vi "Apply Deviation.vi"(8 "error in (no error)":errorcluster, 11 "Tool Path in":refnum<class "Tool Path.lvclass">) -> (0 "error out":errorcluster, 3 "Tool Path out":refnum<class "Tool Path.lvclass">)   [LabVIEW 2019, in "Tool Path.lvclass"]
uses:
  Tool Path.lvclass
  subVIs/typedefs/Schedule Types/Schedule--Formula.ctl
  Settings/Path Settings/Path Settings.lvclass/Path Settings.ctl
  Settings/Path Settings/Path Settings.lvclass
  Settings/ObjectSettings/ObjectSettings.lvclass
  <vilib>/gmath/NI_Gmath.lvlib
  Tool Object/Tool Object.lvclass
panel:
  out "XY Graph":T1(graph)
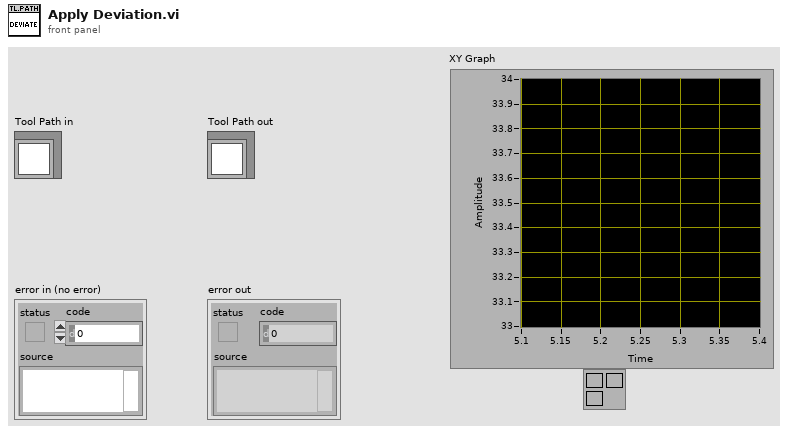
[diagram p1: front panel]
types:
  T1 = cluster{"Resampled X":dbl[], "Resampled Y":dbl[]}[]
  T2 = typedef "Schedule--Formula.ctl" = cluster{"formula":string, "formula length (nm)":dbl, "formula resolution (nm)":dbl}
  T3 = cluster{"Resampled X":dbl[], "Resampled Y":dbl[]}
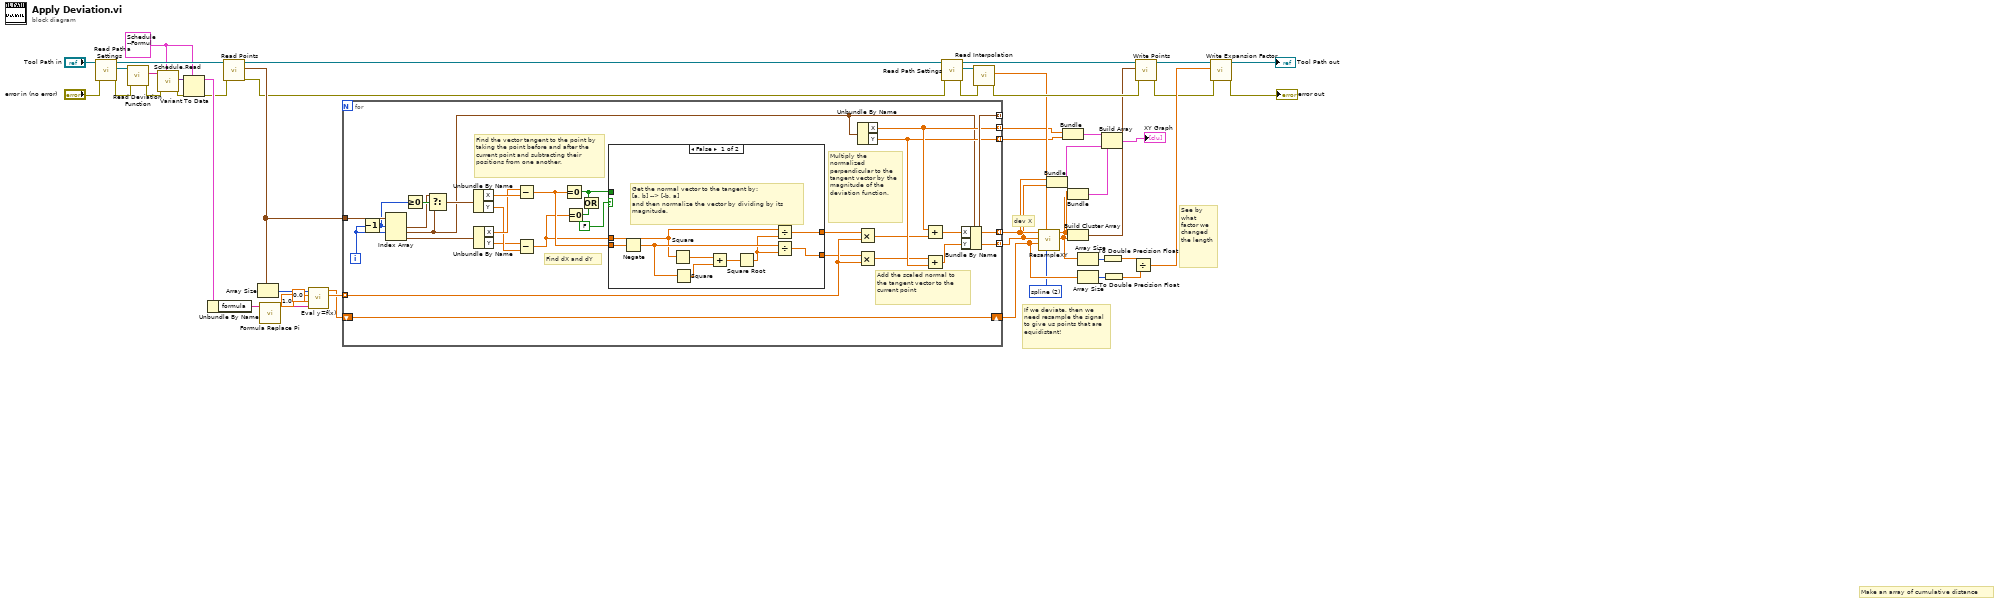
[diagram p0: block diagram]
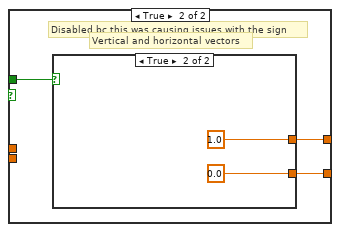
[diagram p2: hidden frame]
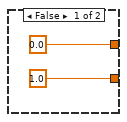
[diagram p3: hidden frame]
diagram:
  w1 = 2 items=["nearest", "linear", "spline", "cubic Hermite", "Lagrange"] ("Interpolation Method")
  w39 = T2 {"formula"="1*(step(170-t)*cos(0.62831853071*t)+step(t-170)*cos(0.62831853071*(t-170))*(-1))", "formula length (nm)"=340.0, "formula resolution (nm)"=0.001} ("Formula")
  # "See by what factor we changed the length"
  # "If we deviate, then we need resample the signal to give us points that are equidistant!"
  # "dev X"
  # "Make an array of cumulative distance"
  n1 = call-dynamic "Read Path Settings.vi"("error in (no error)"="error in (no error)", "Tool Path in"="Tool Path in") -> ("error out"=w38:errorcluster, "Path Settings.lvclass"=w48:refnum<class "Path Settings.lvclass">, "Tool Path out"=w42:refnum<class "Tool Path.lvclass">)  [unwired: 7 in]
  n2 = call-dynamic "Read Deviation Function.vi"("error in (no error)"=w38, "Path Settings in"=w48) -> ("error out"=w28:errorcluster, "Deviation Function"=w45:string)  [unwired: 7 in, 1 out]
  n3 = call "Schedule.Read.vi"("Data to Read"=w39, "error in (no error)"=w28, "Schedule <JSON> In"=w45) -> ("error out"=w44:errorcluster, "Data Out"=w47:variant)  [unwired: 6 in, 1 out]
  n4 = Variant To Data(error in=w44, type=w39, Variant=w47) -> (data=w46:T2, error out=w37:errorcluster)
  n5 = Unbundle By Name(w46) -> ("formula"=w26:string)
  n6 = call-dynamic "Read Points.vi"("error in (no error)"=w37, "Tool Object in"=w42) -> ("error out"=w29:errorcluster, "Points"=w33:cluster{"X":dbl, "Y":dbl}[], "Tool Object out"=w30:refnum<class "Tool Path.lvclass">)  [unwired: 7 in]
  n7 = Array Size(array=w33) -> (size(s)=w34:i32)
  n8 = call "Formula Replace Pi.vi"("Formula In"=w26) -> ("Formula Out"=w25:string)  [unwired: 4 in]
  n9 = call <vilib>:"Eval y=f(x).vi"("formula"=w25, "end"=1.0, "start"=0.0, "number of points"=w34) -> ("Y Values"=w3:dbl[], "X Values"=w2:dbl[])  [unwired: 2 out]
  n10 = for {
    tunnel: w33 -> [w77]
    tunnel: w3 -> [w68] mode=indexing
    tunnel: [w67] -> _ mode=indexing
    tunnel: [w66] -> w5 mode=indexing
    tunnel: [w65] -> w6 mode=indexing
    tunnel: [w64] -> w13 mode=indexing
    tunnel: [w63] -> w12 mode=indexing
    shift-right: [w57] -> w24
    shift-left: w2 -> [w57]
    i -> [w69]
    # "Add the scaled normal to the tangent vector to the current point"
    # "Multiply the normalized perpendicular to the tangent vector by the magnitude of the deviation function."
    # "Find the vector tangent to the point by taking the point before and after the current point and subtracting their positions from one another."
    # "Find dX and dY"
    n11 = Decrement(x=w69) -> (x-1=w62:i32)
    n12 = Index Array(array=w77, index #1=w62, index #2=w69) -> (element #1=w58:cluster{"X":dbl, "Y":dbl}, element #2=w59:cluster{"X":dbl, "Y":dbl}, element #3=w76:cluster{"X":dbl, "Y":dbl})  [unwired: 1 in]
    n13 = Greater Or Equal To 0?(x=w62) -> (x >= 0?=w61:bool)
    n14 = Select(t=w58, s=w61, f=w59) -> (s? t:f=w60:cluster{"X":dbl, "Y":dbl})
    n15 = Unbundle By Name(w60) -> ("X"=w75:dbl, "Y"=w73:dbl)
    n16 = Unbundle By Name(w76) -> ("X"=w74:dbl, "Y"=w72:dbl)
    n17 = Subtract(x=w74, y=w75) -> (x-y=w54:dbl)
    n18 = Subtract(x=w72, y=w73) -> (x-y=w53:dbl)
    n19 = Equal To 0?(x=w54) -> (x = 0?=w70:bool)
    n20 = Equal To 0?(x=w53) -> (x = 0?=w71:bool)
    n21 = Or(x=w70, y=w71) -> ()  [unwired: 1 out]
    n22 = case shown="False" FALSE {
      tunnel: [w79 w87] -> w52
      tunnel: [w85 w88] -> w51
      tunnel: w54 -> [w86 _]
      tunnel: w53 -> [w78 _]
      tunnel: w70 -> [_ w89]
      frame False {
        # "Get the normal vector to the tangent by:\n[a, b] --> [-b, a]\nand then normalize the vector by dividing by its magnitude."
        n23 = Negate(x=w86) -> (-x=w81:dbl)
        n24 = Square(x=w78) -> (x^2=w84:dbl)
        n25 = Square(x=w81) -> (x^2=w83:dbl)
        n26 = Add(x=w84, y=w83) -> (x+y=w82:dbl)
        n27 = Square Root(x=w82) -> (sqrt(x)=w80:dbl)
        n28 = Divide(x=w78, y=w80) -> (x/y=w85:dbl)
        n29 = Divide(x=w81, y=w80) -> (x/y=w79:dbl)
      }
      frame True {
        # "Disabled bc this was causing issues with the sign"
        # "Vertical and horizontal vectors"
        n30 = case shown="True" w89 {
          tunnel: [0.0 1.0] -> w88
          tunnel: [1.0 0.0] -> w87
          frame False {
          }
          frame True {
          }
        }
      }
    }
    n31 = Multiply(x=w51, y=w68) -> (x*y=w56:dbl)
    n32 = Multiply(x=w52, y=w68) -> (x*y=w55:dbl)
    n33 = Unbundle By Name(w59) -> ("X"=w64:dbl, "Y"=w63:dbl)
    n34 = Add(x=w64, y=w56) -> (x+y=w65:dbl)
    n35 = Add(x=w55, y=w63) -> (x+y=w66:dbl)
    n36 = Bundle By Name(cluster=w59, "X"=w65, "Y"=w66) -> (w67:cluster{"X":dbl, "Y":dbl})
  }
  n37 = call-dynamic "Read Path Settings.vi"("error in (no error)"=w29, "Tool Path in"=w30) -> ("error out"=w35:errorcluster, "Path Settings.lvclass"=w36:refnum<class "Path Settings.lvclass">, "Tool Path out"=w32:refnum<class "Tool Path.lvclass">)  [unwired: 7 in]
  n38 = call "Read Interpolation.vi"("error in (no error)"=w35, "Path Settings in"=w36) -> ("error out"=w31:errorcluster, "Interpolation"=w27:dbl)  [unwired: 7 in, 1 out]
  n39 = call "ResampleXY.vi"("Interpolation Method"=w1, "Interpolation Distance"=w27, "t"=w24, "Y"=w5, "X"=w6) -> ("Resampled Y"=w10:dbl[], "Resampled X"=w11:dbl[])  [unwired: 4 in, 1 out]
  n40 = Bundle(w6, w5) -> (w4:cluster{dbl[], dbl[]})  [unwired: 1 in]
  n41 = Bundle(w13, w12) -> (w7:cluster{dbl[], dbl[]})  [unwired: 1 in]
  n42 = Bundle("Resampled X"=w11, "Resampled Y"=w10) -> (w8:T3)  [unwired: 1 in]
  n43 = Build Cluster Array(w11, w10) -> (w9:cluster{"Numeric":dbl, "Numeric":dbl}[])
  n44 = Array Size(array=w10) -> (size(s)=w23:i32)
  n45 = Array Size(array=w24) -> (size(s)=w22:i32)
  n46 = Build Array(w7, w8, w4) -> (→"XY Graph":T1)
  n47 = To Double Precision Float(number=w23) -> (double precision float=w21:dbl)
  n48 = To Double Precision Float(number=w22) -> (double precision float=w20:dbl)
  n49 = Divide(x=w21, y=w20) -> (x/y=w17:dbl)
  n50 = call-dynamic "Write Points.vi"("error in (no error)"=w31, "Points"=w9, "Tool Object in"=w32) -> ("error out"=w16:errorcluster, "Tool Object out"=w19:refnum<class "Tool Path.lvclass">)  [unwired: 7 in]
  n51 = call-dynamic "Write Expansion Factor.vi"("error in (no error)"=w16, "Expansion Factor"=w17, "Tool Path in"=w19) -> ("error out"=→"error out":errorcluster, "Tool Path out"=→"Tool Path out":refnum<class "Tool Path.lvclass">)  [unwired: 7 in]
